vi "Func - VarMan Error Handler (Error Cluster).vi"(7 "InstanceRef":T1, 8 "VarMan VI error in":errorcluster, 9 "error status before":bool, 11 "var name":string) -> (0 "error out":errorcluster, 1 "FuncVI error out":bool, 3 "dup var name":string)   [LabVIEW 2021]
doc: "This VI handles errors returned by VarMan VIs. Refer to the VI help for more details.\n\n<b>error status before</b> control is used to indicate an error occurred before calling a VarMan VI to avoid irrelevant error messages from being added to the CE Error Log.\n\n::: CalcExpress Toolkit :::\nCopyright (c) 2000-2026 Konstantin Shifershteyn. All rights reserved."
uses:
  cetypes.llb/CalcExpress Instance RefNum.ctl
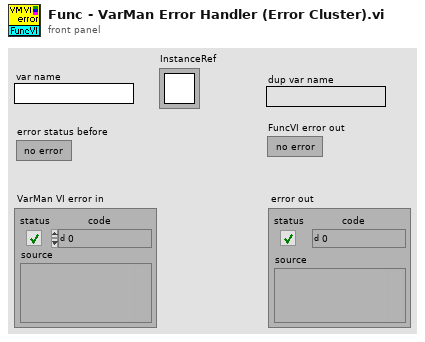
[diagram p1: front panel]
types:
  T1 = typedef "CalcExpress Instance RefNum.ctl" = refnum<k1>
  T2 = typedef "VarMan Error Code.ctl" = u16
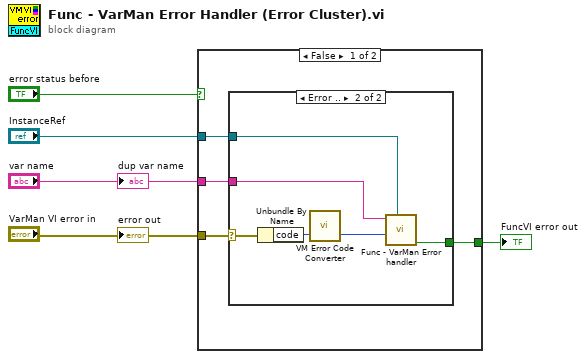
[diagram p0: block diagram]
diagram:
  n1 = case shown="False" "error status before" {
    selector: "error status before" -> [_ w16]
    tunnel: "InstanceRef" -> [w9 _]
    tunnel: "var name" -> [w8 _]
    tunnel: [w7 w16] -> w3
    tunnel: "VarMan VI error in" -> [w6 _]
    frame False {
      n2 = case shown="Error .." w6 {
        selector: w6 -> [_ w14]
        tunnel: w9 -> [_ w12]
        tunnel: [_ w11] -> w7
        tunnel: w8 -> [_ w10]
        frame No Error {
        }
        frame Error {
          n3 = Unbundle By Name(w14) -> ("code"=w15:i32)
          n4 = call "VM Error Code Converter.vi"("VM VI error code in"=w15) -> ("VM Engine error code out"=w13:T2)  [unwired: 1 in, 1 out]
          n5 = call "Func - VarMan Error handler.vi"("InstanceRef"=w12, "VM error code"=w13, "var name"=w10) -> ("error out"=w11:bool)  [unwired: 4 in, 2 out]
        }
      }
    }
    frame True {
    }
  }
  "FuncVI error out" <- w3
  "dup var name" <- "var name"
  "error out" <- "VarMan VI error in"
